vi "Config_Activate_Snapshot.vi"(8 "error in (no error)":errorcluster={"status"=FALSE, "code"=0, "source"="\"\""}, 10 "current mode":string, 11 "Approved ExecutionPlan":string) -> (0 "error out":errorcluster={"status"=FALSE, "code"=0, "source"="\"\""}, 2 "status ok":bool, 3 "Active snapshot ID/handle":string)   [LabVIEW 2026]
doc: "INTENT: Fix active configuration for run. LOGIC: Atomically switch only while idle/ready; record content hash and revision in run record."
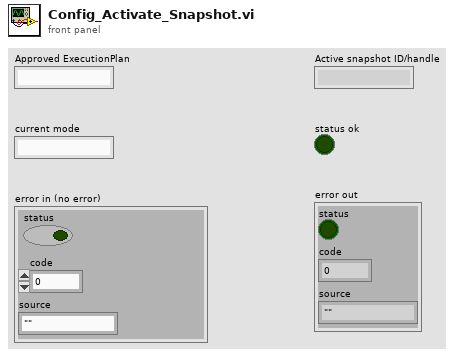
[diagram p1: front panel]
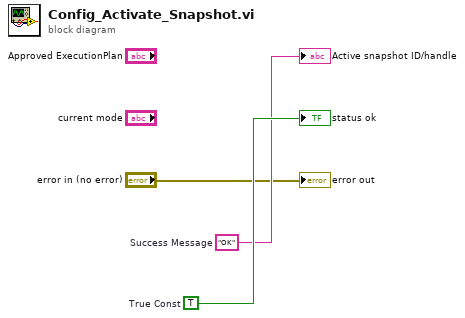
[diagram p0: block diagram]
diagram:
  w3 = TRUE  # True Const
  w2 = "OK"  # Success Message
  "Active snapshot ID/handle" <- w2
  "status ok" <- w3
  "error out" <- "error in (no error)"
